vi "Init.vi"(8 "error in (no error)":errorcluster) -> (0 "error out":errorcluster, 3 "uService out":refnum<class "uService List.lvclass">)   [LabVIEW 2020, in "TALOS.lvlib" / "Classes.lvlib" / "uService List.lvclass"]
uses:
  uService List.lvclass
  uService Properties.ctl
  builds/Actor Framework PPL/Actor Framework.lvlibp/1abvi3w/vi.lib/ActorFramework/Message Enqueuer/Message Enqueuer.lvclass
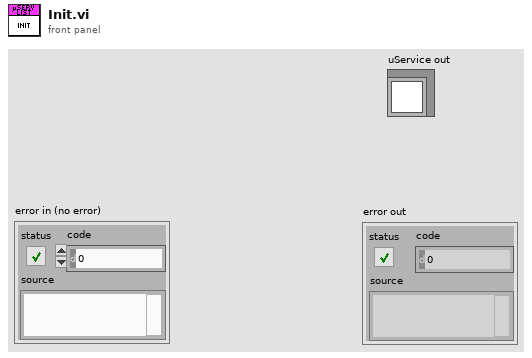
[diagram p1: front panel]
types:
  T1 = typedef "TALOS.lvlib/Classes.lvlib/uService List.lvclass/uService Properties.ctl" = cluster{"uService Queue":refnum<class "Message Enqueuer.lvclass">, "Last Pat":timestamp, "Online":bool, "Vi Ref":refnum<vi>, "Class name":string, "GUI":bool, "FP Items Refs Map":map{string, refnum<vi>}}
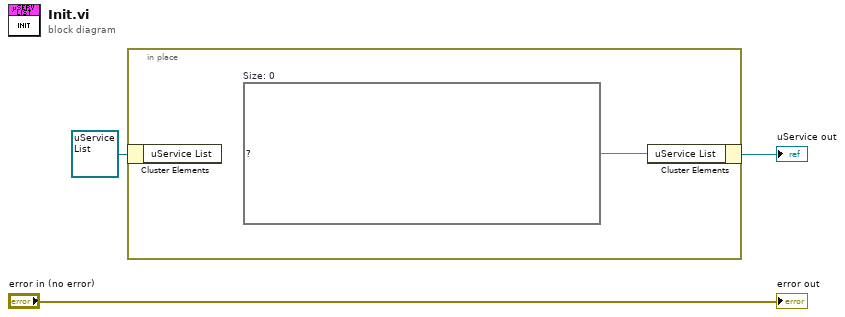
[diagram p0: block diagram]
diagram:
  n1 = in-place {
    w4 = map{string, T1} {}  # Size: 0
    n2 = in-place-cluster #1(refnum<class "uService List.lvclass"> refnum ("uService List")) -> ()  [unwired: 1 out]
    n3 = in-place-cluster #1("uService List"=w4) -> (→"uService out":refnum<class "uService List.lvclass">)
  }
  "error out" <- "error in (no error)"
